vi "Create Connection Handler.vi"(5 "ConnectionHandler in":refnum<class "ConnectionHandler.lvclass">, 8 "error in (no error)":errorcluster, 10 "Connection Configuration":refnum<class "Connection.lvclass">, 11 "Request":refnum<queue>) -> (0 "error out":errorcluster, 3 "ConnectionHandler":refnum<class "ConnectionHandler.lvclass">)   [LabVIEW 2013, in "MQTT Server.lvlib" / "ConnectionHandler.lvclass"]
uses:
  ConnectionHandler.lvclass
  <vilib>/LabVIEW Open Source Project/MQTT Connection/MQTT_Base/Base Class/Request -- cluster.ctl
  <vilib>/LabVIEW Open Source Project/MQTT Control Packets/Control Packets/ControlPacket/ControlPacket.lvclass
  <vilib>/LabVIEW Open Source Project/MQTT Connection/MQTT_Base/Base Class/Response -- cluster.ctl
  <vilib>/LabVIEW Open Source Project/Connection/Connection/Connection.lvclass
  Client Event -- cluster.ctl
  Client Action -- enum.ctl
  ConnectionHandler.lvclass/ConnectionHandler.ctl
  <vilib>/LabVIEW Open Source Project/MQTT Connection/MQTT_Base/Base Class/MQTT_Base.lvclass
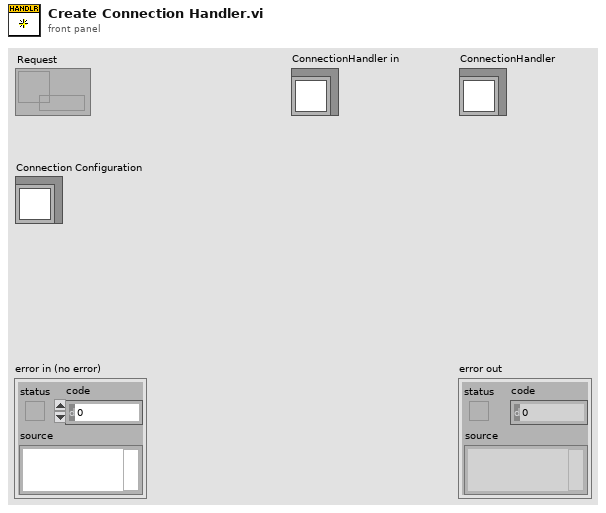
[diagram p1: front panel]
types:
  T1 = typedef "MQTT Server.lvlib/ConnectionHandler.lvclass/Client Event -- cluster.ctl" = cluster{"Action":T2, "Session ID":i32}
  T2 = typedef "MQTT Server.lvlib/ConnectionHandler.lvclass/Client Action -- enum.ctl" = enum16{"Connection", "Disconnection", "Session Stored", "Session Retrieved"}
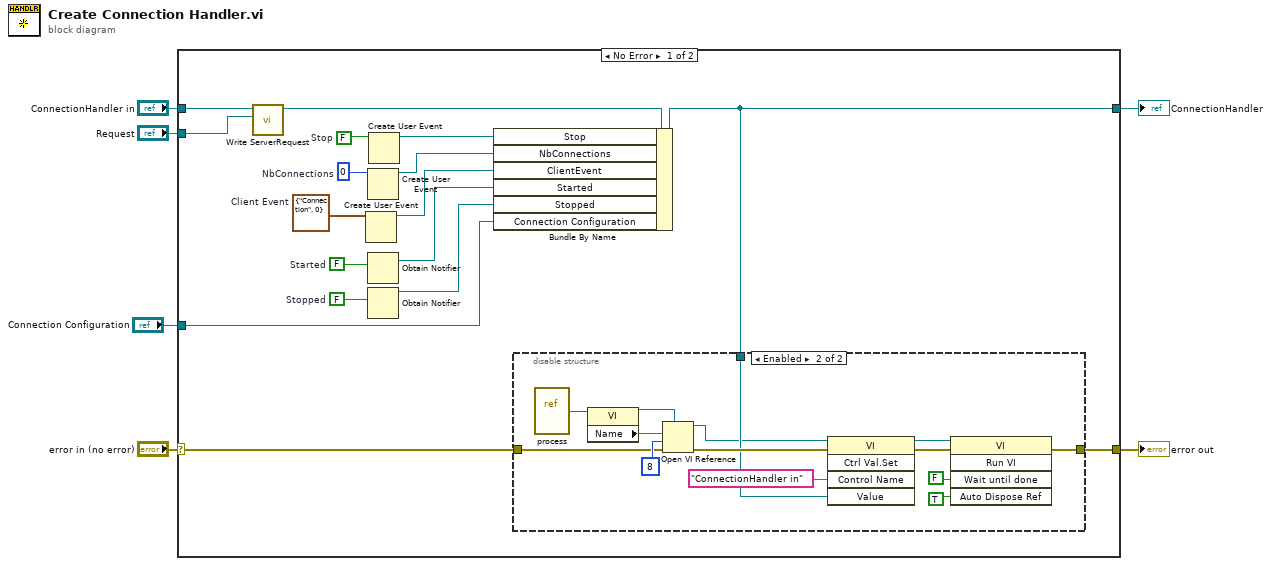
[diagram p0: block diagram]
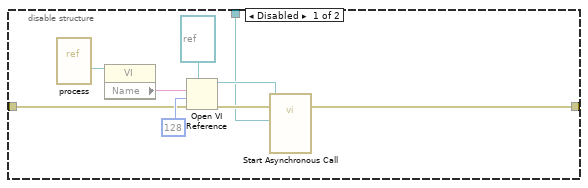
[diagram p2: hidden frame]
diagram:
  n1 = case shown="No Error" "error in (no error)" {
    selector: "error in (no error)" -> [w15 w48]
    tunnel: [w14 w48] -> w5
    tunnel: [w18 w47] -> w3
    tunnel: "ConnectionHandler in" -> [w22 w47]
    tunnel: "Request" -> [w23 _]
    tunnel: "Connection Configuration" -> [w9 _]
    frame No Error {
      w8 = T1 {"Action"=enum."Connection", "Session ID"=0}  # Client Event
      w13 = u32 0  # NbConnections
      w16 = FALSE  # Stopped
      w17 = FALSE  # Started
      w21 = FALSE  # Stop
      n2 = call "Write ServerRequest.vi"("ServerRequest"=w23, "TCPConnectionHandler in"=w22) -> ("TCPConnectionHandler out"=w19:refnum<class "ConnectionHandler.lvclass">)  [unwired: 9 in]
      n3 = Create User Event(user event datatype=w8) -> (user event=w7:refnum<user-event>)  [unwired: 1 in, 1 out]
      n4 = Create User Event(user event datatype=w13) -> (user event=w12:refnum<user-event>)  [unwired: 1 in, 1 out]
      n5 = Obtain Notifier(notification data type=w17) -> (notifier out=w11:refnum<notifier>)  [unwired: 3 in, 2 out]
      n6 = Obtain Notifier(notification data type=w16) -> (notifier out=w10:refnum<notifier>)  [unwired: 3 in, 2 out]
      n7 = Create User Event(user event datatype=w21) -> (user event=w20:refnum<user-event>)  [unwired: 1 in, 1 out]
      n8 = Bundle By Name(cluster=w19, "Stop"=w20, "NbConnections"=w12, "ClientEvent"=w7, "Started"=w11, "Stopped"=w10, "Connection Configuration"=w9) -> (w18:refnum<class "ConnectionHandler.lvclass">)
      n9 = disable-structure shown="Enabled" {
        disable-tunnel: w18 -> [w27 w34]
        disable-tunnel: w15 -> [w26 w35]
        disable-tunnel: [w25 w36] -> w14
        frame Disabled {
          n10 = vi-ref "process.vi"() -> (w32:refnum<vi>)
          n11 = property class="VI"(reference=w32) -> ("Name"=w31:string)  [unwired: 1 in, 2 out]
          n12 = Open VI Reference(type specifier VI Refnum (for type only)=refnum<vi> refnum ("reference out"), vi path=w31, options=128, error in (no error)=w26) -> (vi reference=w30:refnum<vi>, error out=w29:errorcluster)  [unwired: 2 in]
          n13 = call-by-ref "Start Asynchronous Call"(reference=w30, error in=w29, "ConnectionHandler in"=w27) -> (error out=w25:errorcluster)  [unwired: 9 in, 3 out]
        }
        frame Enabled {
          n14 = vi-ref "process.vi"() -> (w37:refnum<vi>)
          n15 = property class="VI"(reference=w37) -> (reference out=w45:refnum<vi>, "Name"=w46:string)  [unwired: 1 in, 1 out]
          n16 = Open VI Reference(type specifier VI Refnum (for type only)=w45, vi path=w46, options=8, error in (no error)=w35) -> (vi reference=w33:refnum<vi>, error out=w39:errorcluster)  [unwired: 2 in]
          n17 = invoke class="VI" method="Ctrl Val.Set"(reference=w33, error in=w39, "Control Name"="ConnectionHandler in", "Value"=w34) -> (reference out=w42:refnum<vi>, error out=w43:errorcluster)  [unwired: 1 in, 3 out]
          n18 = invoke class="VI" method="Run VI"(reference=w42, error in=w43, "Wait until done"=FALSE ("Wait Until Done"), "Auto Dispose Ref"=TRUE ("Auto Dispose Reference")) -> (error out=w36:errorcluster)  [unwired: 1 in, 4 out]
        }
      }
    }
    frame Error {
    }
  }
  "error out" <- w5
  "ConnectionHandler" <- w3
